vi "modbus Tree MCS.vi"() -> (4 "OFF-COIL":T4, 6 "ON-COIL":T3, 8 "Ambietent Left":T1, 10 "Ambient Right":T2)   [LabVIEW 2025]
uses:
  <vilib>/Modbus/master/Modbus Master.lvclass
  <vilib>/Analysis/NI_AALBase.lvlib
  <vilib>/Analysis/baseanly.llb/Mean (DBL).vi
  <vilib>/Modbus/master/Create Master Instance (TCP).vi
panel:
  out "x/y":dbl[](array[numeric])
  out "TREES AVG array":dbl[](array[numeric])
  out "OD_Left side AVG distributed":dbl format="%0.2f"
  out "OD_Right side AVG distributed":dbl format="%0.2f"
  out "ON_Coil AVG distributed":dbl format="%0.2f"
  out "OFF_Coil AVG distributed":dbl format="%0.2f"
  out "AMB LEFT":dbl[](array[numeric])
  out "AMB RIGHT":dbl[](array[numeric])
  out "ON-COIL 2":dbl[](array[numeric])
  out "OFF-COIL 2":dbl[](array[numeric])
  out "error out":errorcluster
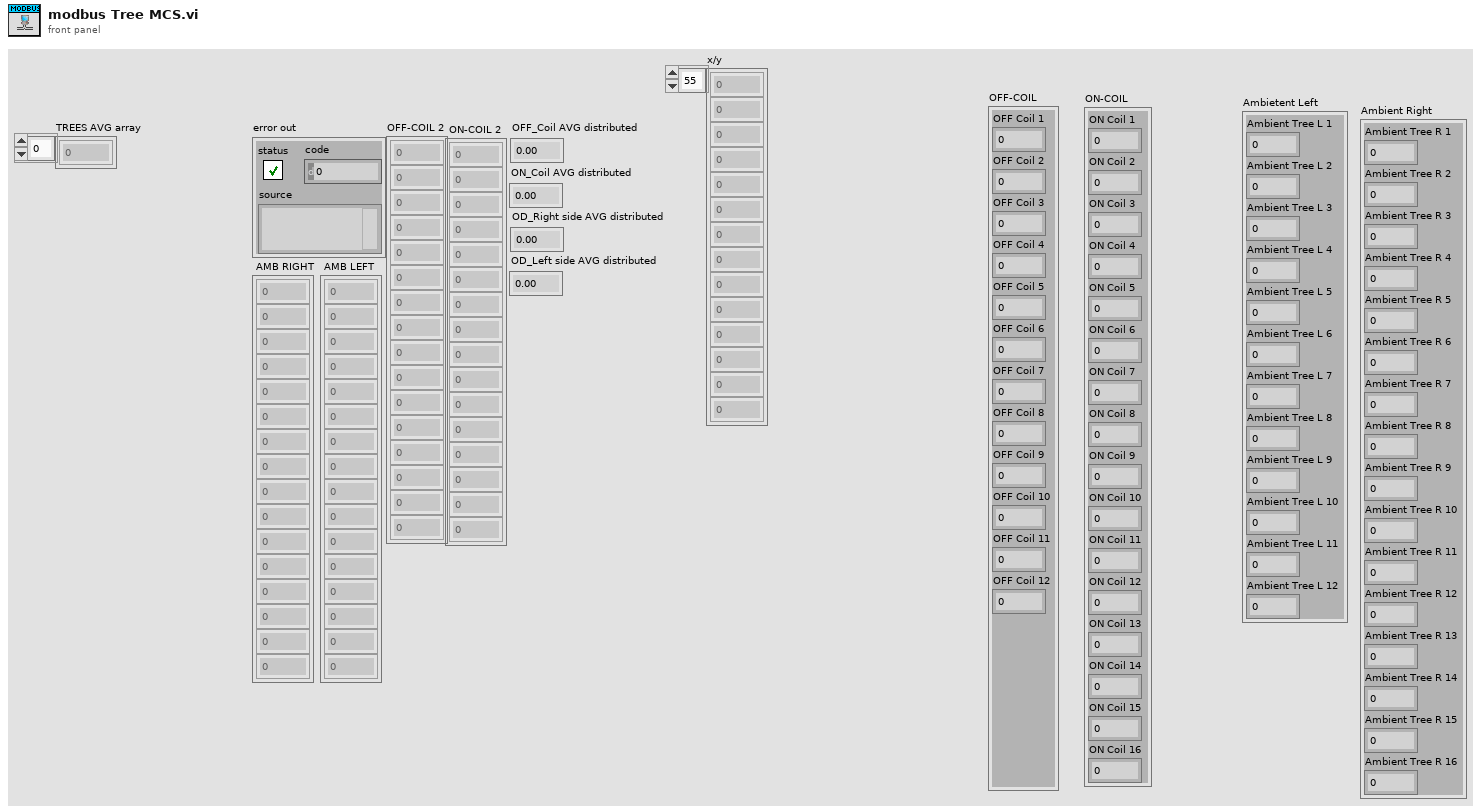
[diagram p1: front panel]
types:
  T1 = cluster{"Ambient Tree L 1":dbl, "Ambient Tree L 2":dbl, "Ambient Tree L 3":dbl, "Ambient Tree L 4":dbl, "Ambient Tree L 5":dbl, "Ambient Tree L 6":dbl, "Ambient Tree L 7":dbl, "Ambient Tree L 8":dbl, "Ambient Tree L 9":dbl, "Ambient Tree L 10":dbl, "Ambient Tree L 11":dbl, "Ambient Tree L 12":dbl}
  T2 = cluster{"Ambient Tree R 1":dbl, "Ambient Tree R 2":dbl, "Ambient Tree R 3":dbl, "Ambient Tree R 4":dbl, "Ambient Tree R 5":dbl, "Ambient Tree R 6":dbl, "Ambient Tree R 7":dbl, "Ambient Tree R 8":dbl, "Ambient Tree R 9":dbl, "Ambient Tree R 10":dbl, "Ambient Tree R 11":dbl, "Ambient Tree R 12":dbl, "Ambient Tree R 13":dbl, "Ambient Tree R 14":dbl, "Ambient Tree R 15":dbl, "Ambient Tree R 16":dbl}
  T3 = cluster{"ON Coil 1":dbl, "ON Coil 2":dbl, "ON Coil 3":dbl, "ON Coil 4":dbl, "ON Coil 5":dbl, "ON Coil 6":dbl, "ON Coil 7":dbl, "ON Coil 8":dbl, "ON Coil 9":dbl, "ON Coil 10":dbl, "ON Coil 11":dbl, "ON Coil 12":dbl, "ON Coil 13":dbl, "ON Coil 14":dbl, "ON Coil 15":dbl, "ON Coil 16":dbl}
  T4 = cluster{"OFF Coil 1":dbl, "OFF Coil 2":dbl, "OFF Coil 3":dbl, "OFF Coil 4":dbl, "OFF Coil 5":dbl, "OFF Coil 6":dbl, "OFF Coil 7":dbl, "OFF Coil 8":dbl, "OFF Coil 9":dbl, "OFF Coil 10":dbl, "OFF Coil 11":dbl, "OFF Coil 12":dbl}
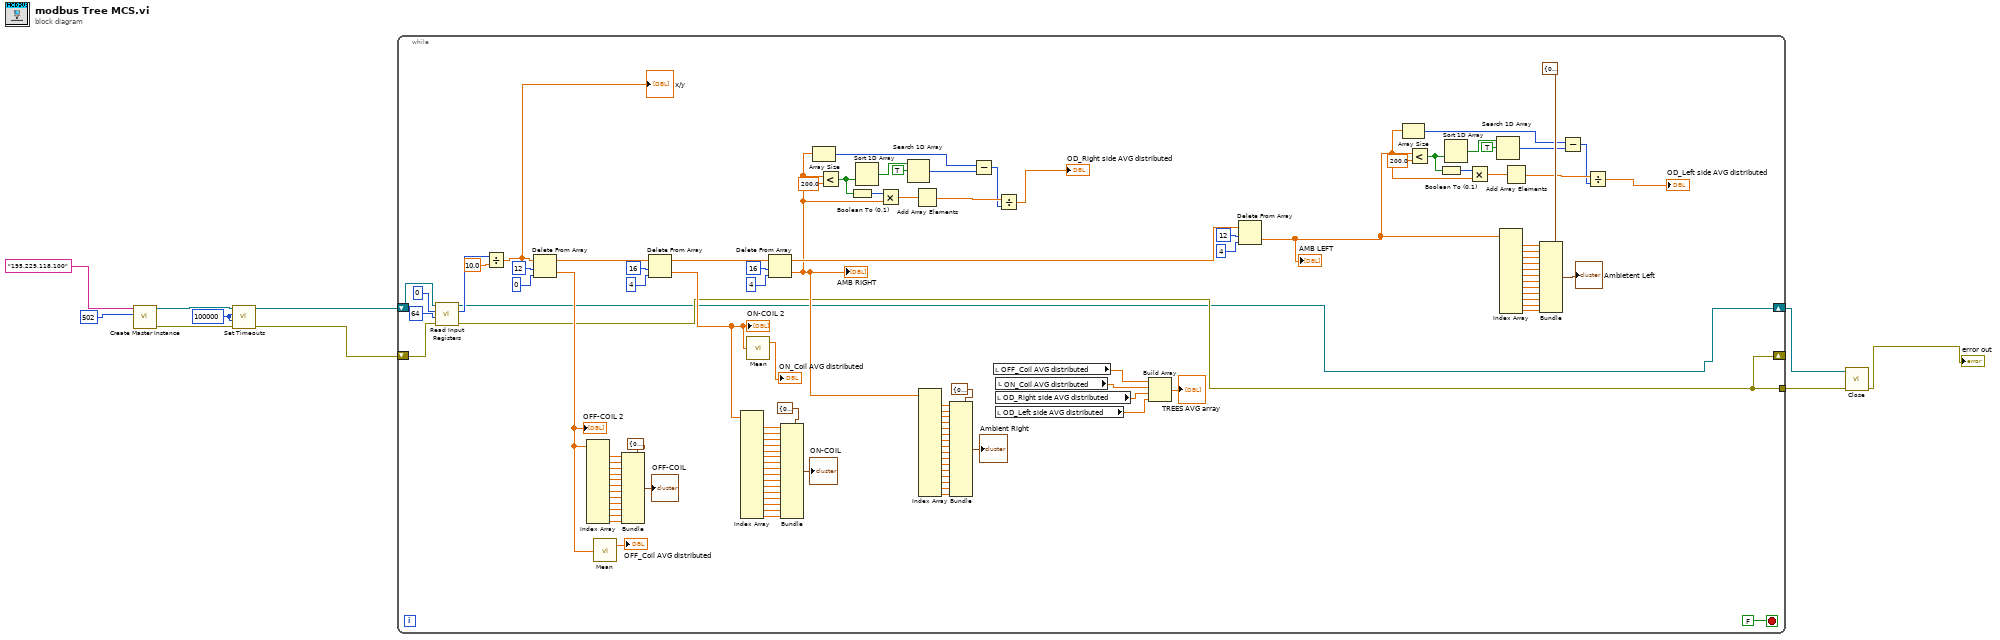
[diagram p0: block diagram]
diagram:
  w4 = 100000 ("read operation timeout (ms)")
  n1 = call-poly <vilib>:"Create Master Instance.vi"("port (502)"=u16 502, "address"="195.229.118.100") -> ("error out"=w5:errorcluster, "TCP master instance"=w6:refnum<class "Modbus Master.lvclass">)  [unwired: 8 in]
  n2 = call <vilib>:"Set Timeouts.vi"("error in (no error)"=w5, "write operation timeout (ms)"=w4, "read operation timeout (ms)"=w4, "Modbus master in"=w6) -> ("error out"=w10:errorcluster, "Modbus master out"=w9:refnum<class "Modbus Master.lvclass">)  [unwired: 6 in]
  n3 = while {
    shift-right: [w13] -> _
    shift-left: w10 -> [w20]
    shift-right: [w12] -> w1
    shift-left: w9 -> [w19]
    tunnel: [w13] -> w3
    stop <- FALSE stop-if-true
    n4 = call-dynamic "Read Input Registers.vi"("error in (no error)"=w20, "number of input registers"=u16 64, "starting address"=u16 0, "Modbus master in"=w19) -> ("error out"=w13:errorcluster, "register values"=w17:u16[], "Modbus master out"=w12:refnum<class "Modbus Master.lvclass">)  [unwired: 5 in]
    n5 = Divide(x=w17, y=10.0) -> (x/y=w11:dbl[])
    "x/y" <- w11
    n6 = Delete From Array(array=w11, length=12, index=0) -> (deleted portion=w115:dbl[], array with subset deleted=w124:dbl[])
    "OFF-COIL 2" <- w115
    n7 = Index Array(array=w115) -> (element #1=w113:dbl, element #2=w112:dbl, element #3=w111:dbl, element #4=w110:dbl, element #5=w109:dbl, element #6=w108:dbl, element #7=w107:dbl, element #8=w106:dbl, element #9=w105:dbl, element #10=w104:dbl, element #11=w103:dbl, element #12=w102:dbl)  [unwired: 12 in]
    n8 = call-poly <vilib>:"Mean.vi"("X"=w115) -> ("mean"=→"OFF_Coil AVG distributed":dbl)  [unwired: 1 out]
    n9 = Bundle(cluster=T4 {"OFF Coil 1"=0.0, "OFF Coil 2"=0.0, "OFF Coil 3"=0.0, "OFF Coil 4"=0.0, "OFF Coil 5"=0.0, "OFF Coil 6"=0.0, "OFF Coil 7"=0.0, "OFF Coil 8"=0.0, "OFF Coil 9"=0.0, "OFF Coil 10"=0.0, "OFF Coil 11"=0.0, "OFF Coil 12"=0.0}, "OFF Coil 1"=w113, "OFF Coil 2"=w112, "OFF Coil 3"=w111, "OFF Coil 4"=w110, "OFF Coil 5"=w109, "OFF Coil 6"=w108, "OFF Coil 7"=w107, "OFF Coil 8"=w106, "OFF Coil 9"=w105, "OFF Coil 10"=w104, "OFF Coil 11"=w103, "OFF Coil 12"=w102) -> (→"OFF-COIL":T4)
    n10 = Delete From Array(array=w124, length=16, index=4) -> (deleted portion=w100:dbl[], array with subset deleted=w121:dbl[])
    "ON-COIL 2" <- w100
    n11 = Index Array(array=w100) -> (element #1=w98:dbl, element #2=w97:dbl, element #3=w96:dbl, element #4=w95:dbl, element #5=w94:dbl, element #6=w93:dbl, element #7=w92:dbl, element #8=w91:dbl, element #9=w90:dbl, element #10=w89:dbl, element #11=w88:dbl, element #12=w87:dbl, element #13=w86:dbl, element #14=w85:dbl, element #15=w84:dbl, element #16=w83:dbl)  [unwired: 16 in]
    n12 = call-poly <vilib>:"Mean.vi"("X"=w100) -> ("mean"=→"ON_Coil AVG distributed":dbl)  [unwired: 1 out]
    n13 = Delete From Array(array=w121, length=16, index=4) -> (deleted portion=w40:dbl[], array with subset deleted=w118:dbl[])
    "AMB RIGHT" <- w40
    n14 = Bundle(cluster=T3 {"ON Coil 1"=0.0, "ON Coil 2"=0.0, "ON Coil 3"=0.0, "ON Coil 4"=0.0, "ON Coil 5"=0.0, "ON Coil 6"=0.0, "ON Coil 7"=0.0, "ON Coil 8"=0.0, "ON Coil 9"=0.0, "ON Coil 10"=0.0, "ON Coil 11"=0.0, "ON Coil 12"=0.0, "ON Coil 13"=0.0, "ON Coil 14"=0.0, "ON Coil 15"=0.0, "ON Coil 16"=0.0}, "ON Coil 1"=w98, "ON Coil 2"=w97, "ON Coil 3"=w96, "ON Coil 4"=w95, "ON Coil 5"=w94, "ON Coil 6"=w93, "ON Coil 7"=w92, "ON Coil 8"=w91, "ON Coil 9"=w90, "ON Coil 10"=w89, "ON Coil 11"=w88, "ON Coil 12"=w87, "ON Coil 13"=w86, "ON Coil 14"=w85, "ON Coil 15"=w84, "ON Coil 16"=w83) -> (→"ON-COIL":T3)
    n15 = Array Size(array=w40) -> (size(s)=w42:i32)
    n16 = Less?(x=w40, y=200.0) -> (x < y?=w39:bool[])
    n17 = Boolean To (0,1)(Boolean=w39) -> (0, 1=w38:i16[])
    n18 = Sort 1D Array(array=w39) -> (sorted array=w44:bool[])
    n19 = Multiply(x=w38, y=w40) -> (x*y=w37:dbl[])
    n20 = Search 1D Array(1D array=w44, element=TRUE) -> (index of element=w41:i32)  [unwired: 1 in]
    n21 = Add Array Elements(numeric array=w37) -> (sum=w36:dbl)
    n22 = Index Array(array=w40) -> (element #1=w80:dbl, element #2=w79:dbl, element #3=w78:dbl, element #4=w77:dbl, element #5=w76:dbl, element #6=w75:dbl, element #7=w74:dbl, element #8=w73:dbl, element #9=w72:dbl, element #10=w71:dbl, element #11=w70:dbl, element #12=w69:dbl, element #13=w68:dbl, element #14=w67:dbl, element #15=w66:dbl, element #16=w65:dbl)  [unwired: 16 in]
    n23 = Bundle(cluster=T2 {"Ambient Tree R 1"=0.0, "Ambient Tree R 2"=0.0, "Ambient Tree R 3"=0.0, "Ambient Tree R 4"=0.0, "Ambient Tree R 5"=0.0, "Ambient Tree R 6"=0.0, "Ambient Tree R 7"=0.0, "Ambient Tree R 8"=0.0, "Ambient Tree R 9"=0.0, "Ambient Tree R 10"=0.0, "Ambient Tree R 11"=0.0, "Ambient Tree R 12"=0.0, "Ambient Tree R 13"=0.0, "Ambient Tree R 14"=0.0, "Ambient Tree R 15"=0.0, "Ambient Tree R 16"=0.0}, "Ambient Tree R 1"=w80, "Ambient Tree R 2"=w79, "Ambient Tree R 3"=w78, "Ambient Tree R 4"=w77, "Ambient Tree R 5"=w76, "Ambient Tree R 6"=w75, "Ambient Tree R 7"=w74, "Ambient Tree R 8"=w73, "Ambient Tree R 9"=w72, "Ambient Tree R 10"=w71, "Ambient Tree R 11"=w70, "Ambient Tree R 12"=w69, "Ambient Tree R 13"=w68, "Ambient Tree R 14"=w67, "Ambient Tree R 15"=w66, "Ambient Tree R 16"=w65) -> (→"Ambient Right":T2)
    n24 = Subtract(x=w42, y=w41) -> (x-y=w35:i32)
    n25 = local read "OFF_Coil AVG distributed"() -> (w50:dbl)
    n26 = local read "OD_Right side AVG distributed"() -> (w48:dbl)
    n27 = local read "OD_Left side AVG distributed"() -> (w47:dbl)
    n28 = local read "ON_Coil AVG distributed"() -> (w49:dbl)
    n29 = Divide(x=w36, y=w35) -> (x/y=→"OD_Right side AVG distributed":dbl)
    n30 = Build Array(w50, w49, w48, w47) -> (→"TREES AVG array":dbl[])
    n31 = Delete From Array(array=w118, length=12, index=4) -> (deleted portion=w23:dbl[])  [unwired: 1 out]
    "AMB LEFT" <- w23
    n32 = Array Size(array=w23) -> (size(s)=w30:i32)
    n33 = Less?(x=w23, y=200.0) -> (x < y?=w28:bool[])
    n34 = Boolean To (0,1)(Boolean=w28) -> (0, 1=w27:i16[])
    n35 = Sort 1D Array(array=w28) -> (sorted array=w32:bool[])
    n36 = Multiply(x=w27, y=w23) -> (x*y=w26:dbl[])
    n37 = Search 1D Array(1D array=w32, element=TRUE) -> (index of element=w29:i32)  [unwired: 1 in]
    n38 = Index Array(array=w23) -> (element #1=w62:dbl, element #2=w61:dbl, element #3=w60:dbl, element #4=w59:dbl, element #5=w58:dbl, element #6=w57:dbl, element #7=w56:dbl, element #8=w55:dbl, element #9=w54:dbl, element #10=w53:dbl, element #11=w52:dbl, element #12=w51:dbl)  [unwired: 12 in]
    n39 = Add Array Elements(numeric array=w26) -> (sum=w25:dbl)
    n40 = Bundle(cluster=T1 {"Ambient Tree L 1"=0.0, "Ambient Tree L 2"=0.0, "Ambient Tree L 3"=0.0, "Ambient Tree L 4"=0.0, "Ambient Tree L 5"=0.0, "Ambient Tree L 6"=0.0, "Ambient Tree L 7"=0.0, "Ambient Tree L 8"=0.0, "Ambient Tree L 9"=0.0, "Ambient Tree L 10"=0.0, "Ambient Tree L 11"=0.0, "Ambient Tree L 12"=0.0}, "Ambient Tree L 1"=w62, "Ambient Tree L 2"=w61, "Ambient Tree L 3"=w60, "Ambient Tree L 4"=w59, "Ambient Tree L 5"=w58, "Ambient Tree L 6"=w57, "Ambient Tree L 7"=w56, "Ambient Tree L 8"=w55, "Ambient Tree L 9"=w54, "Ambient Tree L 10"=w53, "Ambient Tree L 11"=w52, "Ambient Tree L 12"=w51) -> (→"Ambietent Left":T1)
    n41 = Subtract(x=w30, y=w29) -> (x-y=w24:i32)
    n42 = Divide(x=w25, y=w24) -> (x/y=→"OD_Left side AVG distributed":dbl)
  }
  n43 = call-dynamic "Close.vi"("error in (no error)"=w3, "Modbus master in"=w1) -> ("error out"=→"error out":errorcluster)  [unwired: 9 in]
